vi "Actor Core.vi"(8 "error in":cluster{"状态":bool, "代码":i32, "源":string} caption="错误输入", 11 "JOY in":refnum<class "JoyStick.lvclass">) -> (0 "error out":cluster{"状态":bool, "代码":i32, "源":string} caption="错误输出", 3 "操作者输出":refnum<class "Actor.lvclass">)   [LabVIEW 2014, in "JoyStick.lvlib" / "JoyStick.lvclass"]
doc: "Actor Core.vi包含操作者的主要消息处理循环。操作者通常位于该循环中，在各种消息到达时对消息进行处理。如Do.vi消息返回任何错误，该循环将停止运行，错误代码43将被作为“无错误停止”的标准信号发送给调用方。如需更改上述行为，可在子孙类的Handle Error.vi中对该部分逻辑进行重写。"
uses:
  JoyStick.lvclass
  <vilib>/ActorFramework/Actor/Actor.lvclass
  <vilib>/MakerHub/Xbox-One-Controller/Private/Type Defs/Indicators/All Buttons Visual.ctl
  <vilib>/MakerHub/Xbox-One-Controller/Private/Type Defs/Indicators/A.ctl
  <vilib>/MakerHub/Xbox-One-Controller/Private/Type Defs/Indicators/B.ctl
  <vilib>/MakerHub/Xbox-One-Controller/Private/Type Defs/Indicators/X.ctl
  <vilib>/MakerHub/Xbox-One-Controller/Private/Type Defs/Indicators/Y.ctl
  <vilib>/MakerHub/Xbox-One-Controller/Private/Type Defs/Indicators/Left Bumper.ctl
  <vilib>/MakerHub/Xbox-One-Controller/Private/Type Defs/Indicators/Right Bumper.ctl
  <vilib>/MakerHub/Xbox-One-Controller/Private/Type Defs/Indicators/View.ctl
  <vilib>/MakerHub/Xbox-One-Controller/Private/Type Defs/Indicators/Menu.ctl
  <vilib>/MakerHub/Xbox-One-Controller/Private/Type Defs/Indicators/Thumbstick.ctl
  <vilib>/MakerHub/Xbox-One-Controller/Private/Type Defs/Indicators/All Axis Data.ctl
  <vilib>/MakerHub/Xbox-One-Controller/Private/Type Defs/Indicators/DPad Enum.ctl
  <vilib>/ActorFramework/Actor/Actor.lvclass/Actor.ctl
  JoyStick.lvclass/JoyStick.ctl
  <vilib>/ActorFramework/Message Enqueuer/Message Enqueuer.lvclass/Message Enqueuer.ctl
  <vilib>/ActorFramework/Message Enqueuer/Enqueue.vi
  <vilib>/MakerHub/Xbox-One-Controller/Public/Open First Controller.vi
  <vilib>/ActorFramework/Message Priority Queue/Priority Enqueue.vi
  Wrapper_lib/zsActor/ActorWrapper.lvclass
  <vilib>/MakerHub/Xbox-One-Controller/LMH-Xbox-One-Controller.lvlib
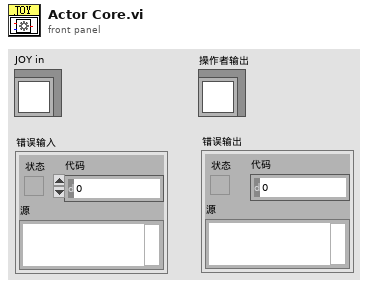
[diagram p1: front panel]
types:
  T1 = typedef "LMH-Xbox-One-Controller.lvlib/All Buttons Visual.ctl" = cluster{"A":T2, "B":T3, "X":T4, "Y":T5, "Left Bumper":T6, "Right Bumper":T7, "View Button":T8, "Menu Button":T9, "Left Stick":T10, "Right Stick":T10}
  T2 = typedef "LMH-Xbox-One-Controller.lvlib/A.ctl" = bool
  T3 = typedef "LMH-Xbox-One-Controller.lvlib/B.ctl" = bool
  T4 = typedef "LMH-Xbox-One-Controller.lvlib/X.ctl" = bool
  T5 = typedef "LMH-Xbox-One-Controller.lvlib/Y.ctl" = bool
  T6 = typedef "LMH-Xbox-One-Controller.lvlib/Left Bumper.ctl" = bool
  T7 = typedef "LMH-Xbox-One-Controller.lvlib/Right Bumper.ctl" = bool
  T8 = typedef "LMH-Xbox-One-Controller.lvlib/View.ctl" = bool
  T9 = typedef "LMH-Xbox-One-Controller.lvlib/Menu.ctl" = bool
  T10 = typedef "LMH-Xbox-One-Controller.lvlib/Thumbstick.ctl" = bool
  T11 = typedef "LMH-Xbox-One-Controller.lvlib/All Axis Data.ctl" = cluster{"Left Stick":cluster{"X Axis":i32, "Y Axis":i32}, "Right Stick":cluster{"X Axis":i32, "Y Axis":i32}, "Triggers":i32, "D-Pad":T12}
  T12 = typedef "LMH-Xbox-One-Controller.lvlib/DPad Enum.ctl" = enum16{"Idle", "Up", "Up / Right", "Right", "Down / Right", "Down", "Down / Left", "Left", "Up / Left"}
  T13 = typedef "LMH-Xbox-One-Controller.lvlib/Xbox One Controller Ref.ctl" = cluster{"Controller Ref":refnum<k1>, "Event Refnum":refnum<event-registration>, "Worker Ref":refnum<vi>}
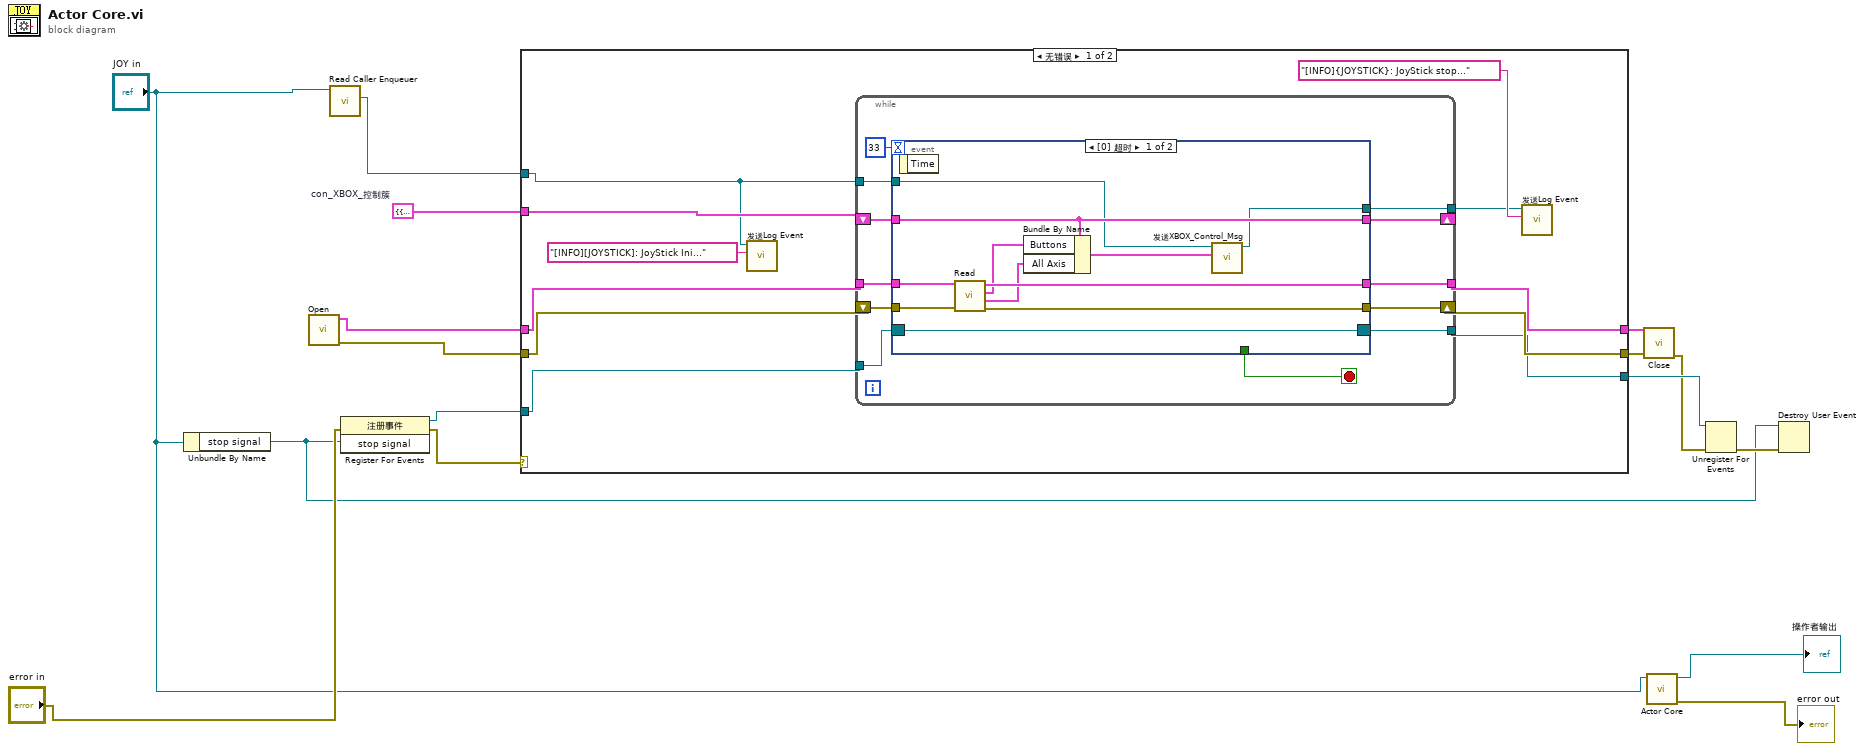
[diagram p0: block diagram]
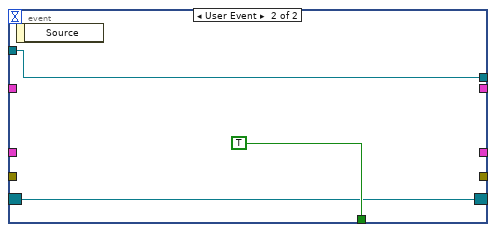
[diagram p2: hidden frame]
diagram:
  w10 = cluster{"Buttons":T1, "All Axis":T11} {"Buttons"={"A"=FALSE, "B"=FALSE, "X"=FALSE, "Y"=FALSE, "Left Bumper"=FALSE, "Right Bumper"=FALSE, "View Button"=FALSE, "Menu Button"=FALSE, "Left Stick"=FALSE, "Right Stick"=FALSE}, "All Axis"={"Left Stick"={"X Axis"=0, "Y Axis"=0}, "Right Stick"={"X Axis"=0, "Y Axis"=0}, "Triggers"=0, "D-Pad"=enum."Idle"}}  # con_XBOX_控制簇
  n1 = Unbundle By Name("JOY in") -> ("stop signal"=w1:refnum<user-event>)
  n2 = call-poly <vilib>:"Open.vi"() -> ("Error Out"=w12:errorcluster, "Xbox One Controller"=w11:T13)  [unwired: 9 in, 1 out]
  n3 = call <vilib>:"Read Caller Enqueuer.vi"("Actor"="JOY in") -> ("Caller Enqueuer"=w9:refnum<class "Message Enqueuer.lvclass">)  [unwired: 10 in]
  n4 = register-events(error in="error in", w1) -> (reference out=w6:refnum<event-registration>, error out=w8:errorcluster)  [unwired: 1 in]
  n5 = case shown="无错误" w8 {
    tunnel: [w27 w56] -> w14
    tunnel: [w26 w55] -> w13
    tunnel: w12 -> [w25 w55]
    tunnel: w11 -> [w24 w56]
    tunnel: w10 -> [w23 _]
    tunnel: w9 -> [w19 _]
    tunnel: w6 -> [w22 w54]
    tunnel: [w21 w54] -> w5
    frame No Error {
      n6 = call "发送Log Event.vi"("Event Text"="[INFO][JOYSTICK]: JoyStick Ini...", "消息待入队列"=w19) -> ()  [unwired: 8 in, 2 out]
      n7 = while {
        shift-right: [w35] -> w26
        shift-left: w25 -> [w38]
        tunnel: w24 -> [w39]
        tunnel: [w37] -> w27
        tunnel: w19 -> [w33]
        shift-right: [w32] -> _
        shift-left: w23 -> [w34]
        tunnel: w22 -> [w31]
        tunnel: [w29] -> w21
        tunnel: [w28] -> w17
        stop <- w30 stop-if-true
        n8 = event shown="[0] 超时" {
          selector: w31 -> [w43 w52]
          dyn-events: [w43 w52] -> w29
          timeout: 33 -> [_ _]
          tunnel: w39 -> [w50 _]
          tunnel: w38 -> [w49 _]
          tunnel: [w48 _] -> w35
          tunnel: [w47 _] -> w37
          tunnel: w34 -> [w46 _]
          tunnel: w33 -> [w41 w51]
          tunnel: [w46 _] -> w32
          tunnel: [_ TRUE] -> w30
          tunnel: [w40 w51] -> w28
          event Timeout {
            n9 = event-data() -> ()  [unwired: 1 in, 1 out]
            n10 = call <vilib>:"Read.vi"("Error In"=w49, "Xbox One Controller Ref"=w50) -> ("Error Out"=w48:errorcluster, "All Axis"=w44:T11, "Buttons"=w45:T1, "Xbox One Controller Ref"=w47:T13)  [unwired: 6 in]
            n11 = Bundle By Name(cluster=w46, "Buttons"=w45, "All Axis"=w44) -> (w42:cluster{"Buttons":T1, "All Axis":T11})
            n12 = call "发送XBOX_Control_Msg.vi"("XBOX_Control"=w42, "消息待入队列"=w41) -> ("消息待入队列输出"=w40:refnum<class "Message Enqueuer.lvclass">)  [unwired: 8 in, 1 out]
          }
          event User Event {
            n13 = event-data() -> ()  [unwired: 1 in, 1 out]
          }
        }
      }
      n14 = call "发送Log Event.vi"("Event Text"="[INFO]{JOYSTICK}: JoyStick stop...", "消息待入队列"=w17) -> ()  [unwired: 8 in, 2 out]
    }
    frame Error {
    }
  }
  n15 = call <vilib>:"Close.vi"("Error In"=w13, "Xbox One Controller Ref"=w14) -> ("Error Out"=w4:errorcluster)  [unwired: 9 in]
  n16 = call-parent "Actor Core.vi"("Actor in"="JOY in") -> ("error out"=→"error out":errorcluster, "Actor out"=→"操作者输出":refnum<class "Actor.lvclass">)  [unwired: 9 in]
  n17 = Unregister For Events(event registration refnum=w5, error in=w4) -> (error out=w7:errorcluster)
  n18 = Destroy User Event(user event=w1, error in=w7) -> ()  [unwired: 1 out]
